vi "lvmcp_relabel.vi"() -> ()   [LabVIEW 2015]
panel:
  out "error out":errorcluster
  in  "text":string
  in  "reference":refnum<vi>
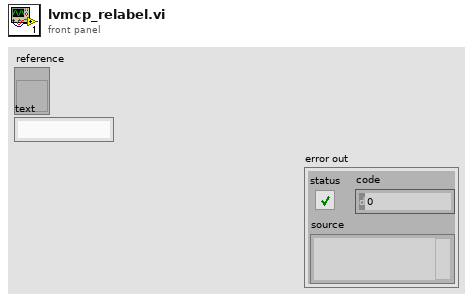
[diagram p1: front panel]
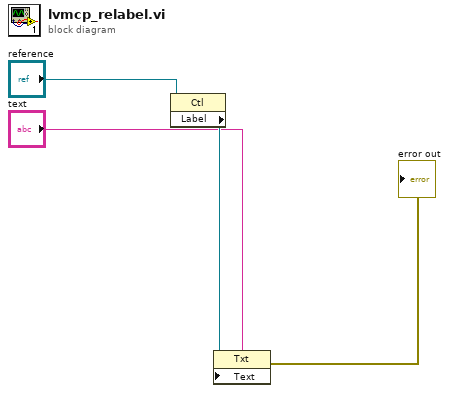
[diagram p0: block diagram]
diagram:
  n1 = property class="Ctl"(reference="reference") -> (error out=w2:errorcluster, "Label"=w4:refnum<vi>)  [unwired: 1 in, 1 out]
  n2 = property class="Txt"(reference=w4, error in=w2, "Text"="text") -> (error out=→"error out":errorcluster)  [unwired: 1 out]
